vi "Save Package For Previous.vi"(8 "error in (no error)":errorcluster, 10 "LabVIEW Version":string="20.0", 11 "Package File":path) -> (0 "error out":errorcluster, 2 "Re-saved Files":string)   [LabVIEW 2020]
doc: "Unpacks a built VI package, re-saves every VI/control in it that is not saved in LabVIEW Version (Save For Previous), and repacks it in place.\n\nWorkaround for VIPM occasionally saving VIs that contain VIM instances in an intermediate LabVIEW version instead of the build spec's save version. Meant to be called from the VIPM Post-Build action: VIPM computes the package ID after that action, so the repacked package still installs.\n\nFiles whose version cannot be read (non-VI files) are left untouched. Re-saved Files lists the paths that were re-saved, one per line."
uses:
  vipm-package-building-extensions/vi_package_building_extensions.lvlib
  31e72c73-b8e8-4e4e-b268-7c3210cc91d9.vi
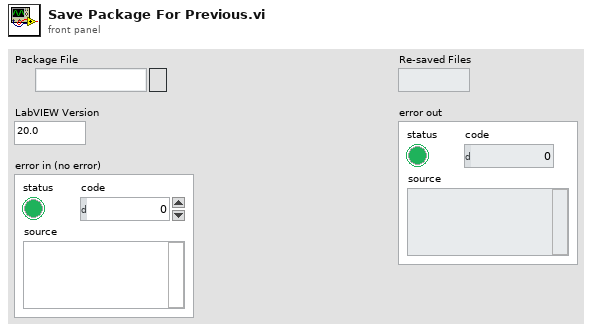
[diagram p1: front panel]
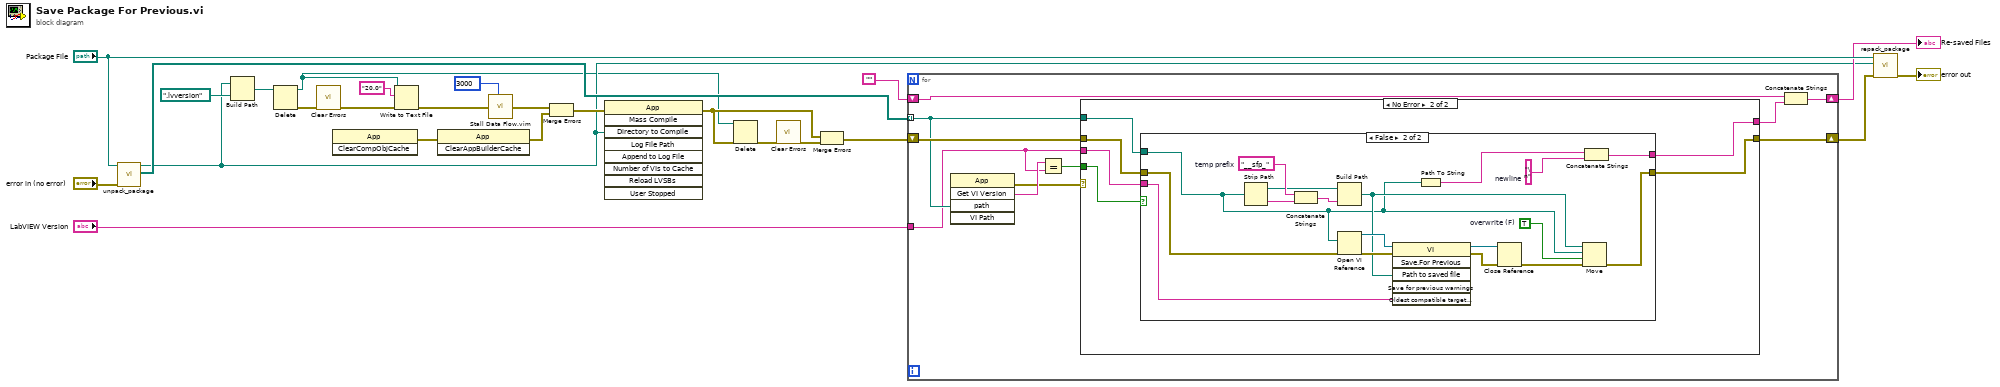
[diagram p0: block diagram]
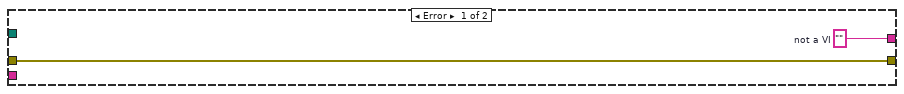
[diagram p2: hidden frame]
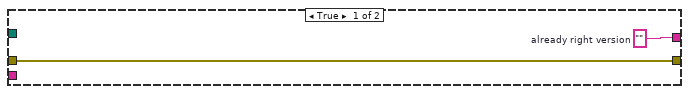
[diagram p3: hidden frame]
diagram:
  n1 = call "unpack_package.vi"("error in (no error)"="error in (no error)", "Package File"="Package File") -> ("Unpacked Files"=w24:path[], "Unpacked Package Directory"=w3:path)  [unwired: 7 in, 1 out]
  n2 = Build Path(base path=w3, name or relative path=path ".lvversion") -> (appended path=w15:path)
  n3 = Delete(path (use dialog)=w15) -> (deleted path=w1:path, error out=w14:errorcluster)  [unwired: 4 in, 1 out]
  n4 = call <vilib>:"Clear Errors.vi"("error in (no error)"=w14) -> ("error out"=w13:errorcluster)  [unwired: 5 in, 1 out]
  n5 = invoke class="App" method="ClearCompObjCache"() -> (error out=w17:errorcluster)  [unwired: 3 in, 2 out]
  n6 = Write to Text File(file (use dialog)=w1, text="20.0", error in=w13) -> (error out=w11:errorcluster)  [unwired: 1 in, 2 out]
  n7 = invoke class="App" method="ClearAppBuilderCache"(error in=w17) -> (error out=w9:errorcluster)  [unwired: 2 in, 2 out]
  n8 = call "Stall Data Flow.vim"("value in"=w11, "milliseconds to wait"=u32 3000) -> ("value out"=w7:errorcluster)  [unwired: 1 out]
  n9 = Merge Errors(w7, w9) -> (w10:errorcluster)
  n10 = invoke class="App" method="Mass Compile"(error in=w10, "Directory to Compile"=w3) -> (error out=w8:errorcluster)  [unwired: 7 in, 8 out]
  n11 = Delete(path (use dialog)=w1, error in=w8) -> (error out=w4:errorcluster)  [unwired: 3 in, 2 out]
  n12 = call <vilib>:"Clear Errors.vi"("error in (no error)"=w4) -> ("error out"=w5:errorcluster)  [unwired: 5 in, 1 out]
  n13 = Merge Errors(w8, w5) -> (w2:errorcluster)
  n14 = for {
    tunnel: w24 -> [w32] mode=indexing
    tunnel: "LabVIEW Version" -> [w31]
    shift-right: [w30] -> w21
    shift-left: w2 -> [w34]
    shift-right: [w27] -> w20
    shift-left: "" -> [w26]
    n15 = invoke class="App" method="Get VI Version"("path"=w32) -> (error out=w29:errorcluster, "GetVIVers"=w35:string)  [unwired: 4 in, 3 out]
    n16 = Equal?(x=w35, y=w31) -> (x = y?=w33:bool)
    n17 = case shown="No Error" w29 {
      tunnel: w34 -> [w37 w43]
      tunnel: w33 -> [_ w40]
      tunnel: w32 -> [_ w42]
      tunnel: w31 -> [_ w41]
      tunnel: [w37 w39] -> w30
      tunnel: [w36 w38] -> w28
      frame Error {
        w36 = ""  # not a VI
      }
      frame No Error {
        n18 = case shown="False" w40 {
          tunnel: w43 -> [w45 w59]
          tunnel: w42 -> [_ w50]
          tunnel: w41 -> [_ w56]
          tunnel: [w45 w47] -> w39
          tunnel: [w44 w46] -> w38
          frame True {
            w44 = ""  # already right version
          }
          frame False {
            w48 = "\n"  # newline
            w52 = TRUE  # overwrite (F)
            w63 = "__sfp_"  # temp prefix
            n19 = Strip Path(path=w50) -> (stripped path=w61:path, name=w62:string)
            n20 = Concatenate Strings(w63, w62) -> (w60:string)
            n21 = Build Path(base path=w61, name or relative path=w60) -> (appended path=w53:path)
            n22 = Open VI Reference(vi path=w50, error in (no error)=w59) -> (vi reference=w58:refnum<vi>, error out=w57:errorcluster)  [unwired: 4 in]
            n23 = invoke class="VI" method="Save.For Previous"(reference=w58, error in=w57, "Path to saved file"=w53, "Oldest compatible target version"=w56) -> (reference out=w55:refnum<vi>, error out=w54:errorcluster)  [unwired: 2 in, 4 out]
            n24 = Path To String(path=w50) -> (string=w49:string)
            n25 = Close Reference(reference=w55, error in (no error)=w54) -> (error out=w51:errorcluster)
            n26 = Move(source path=w53, error in=w51, 9:w52, 10:w50) -> (error out=w47:errorcluster)  [unwired: 1 in, 2 out]
            n27 = Concatenate Strings(w49, w48) -> (w46:string)
          }
        }
      }
    }
    n28 = Concatenate Strings(w26, w28) -> (w27:string)
  }
  "Re-saved Files" <- w20
  n29 = call "repack_package.vi"("error in (no error)"=w21, "Unpacked Package Directory"=w3, "Package File"="Package File") -> ("error out"=→"error out":errorcluster)  [unwired: 8 in]
